vi "VIH Project Tree - Is Drop Allowed.vi"(8 "error in":errorcluster, 9 "Target Item Tag":string, 10 "Source Item Tags":string[](array[string]), 11 "Tree Refnum":refnum<vi>) -> (0 "error out":errorcluster, 1 "Drop Allowed":bool, 3 "dup Tree Refnum":refnum<vi>)   [LabVIEW 2014]
doc: "::: VI Helpeks :::\nCopyright (c) 2000-2026 Konstantin Shifershteyn. All rights reserved."
panel:
  # "VI Helpeks\nCopyright (c) 2012-2026 Konstantin Shifershteyn"
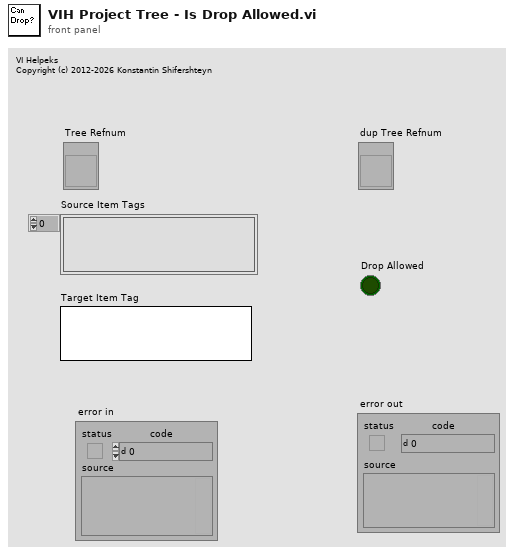
[diagram p1: front panel]
types:
  T1 = typedef "VIH Project Tree Typedef - Tree Item Type.ctl" = enum32{"<Invalid>", "Project", "Proj Files", "Proj Rules", "File Group", "Rule Group", "Any File", "LV Func", ".mnu", ".mnu (dyn)", ".vi", ".vi (dyn)", ".vit", ".vit (dyn)", ".ctl", ".ctl (dyn)", ".ctt", ".ctt (dyn)", "polyVI", "polyVI (dyn)", "expVI", "expVI (dyn)", "HTML", "PolyVI Inst"}
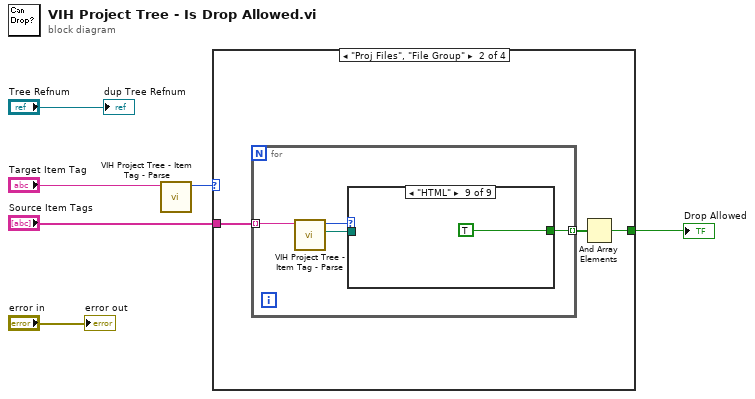
[diagram p0: block diagram]
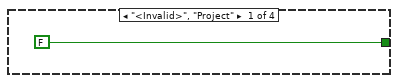
[diagram p2: hidden frame]
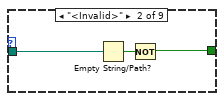
[diagram p4: hidden frame]
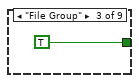
[diagram p5: hidden frame]
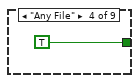
[diagram p6: hidden frame]
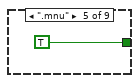
[diagram p7: hidden frame]
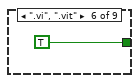
[diagram p8: hidden frame]
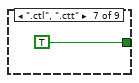
[diagram p9: hidden frame]
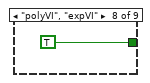
[diagram p10: hidden frame]
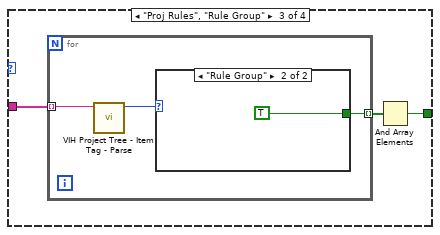
[diagram p11: hidden frame]
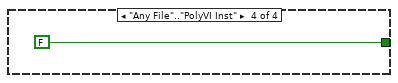
[diagram p13: hidden frame]
diagram:
  n1 = call "VIH Project Tree - Item Tag - Parse.vi"("Tree Item Tag"="Target Item Tag") -> ("Item Type"=w2:T1)  [unwired: 8 in, 2 out]
  n2 = case shown="\"Proj Files\", \"File Group\"" w2 {
    tunnel: [FALSE w9 w26 FALSE] -> w6
    tunnel: "Source Item Tags" -> [_ w8 w25 _]
    frame "<Invalid>", "Project" {
    }
    frame "Proj Files", "File Group" {
      n3 = for {
        tunnel: [w14] -> w10 mode=indexing
        tunnel: w8 -> [w13] mode=indexing
        n4 = call "VIH Project Tree - Item Tag - Parse.vi"("Tree Item Tag"=w13) -> ("Item File Path"=w11:path, "Item Type"=w12:T1)  [unwired: 8 in, 1 out]
        n5 = case shown="\"HTML\"" w12 {
          tunnel: [_ w16 TRUE TRUE TRUE TRUE TRUE TRUE TRUE] -> w14
          tunnel: w11 -> [_ w15 _ _ _ _ _ _ _]
          frame Default {
          }
          frame "<Invalid>" {
            n6 = Empty String/Path?(string/path=w15) -> (empty?=w17:bool)
            n7 = Not(x=w17) -> (.not. x?=w16:bool)
          }
          frame "File Group" {
          }
          frame "Any File" {
          }
          frame ".mnu" {
          }
          frame ".vi", ".vit" {
          }
          frame ".ctl", ".ctt" {
          }
          frame "polyVI", "expVI" {
          }
          frame "HTML" {
          }
        }
      }
      n8 = And Array Elements(Boolean array=w10) -> (logical AND=w9:bool)
    }
    frame "Proj Rules", "Rule Group" {
      n9 = for {
        tunnel: [w30] -> w27 mode=indexing
        tunnel: w25 -> [w29] mode=indexing
        n10 = call "VIH Project Tree - Item Tag - Parse.vi"("Tree Item Tag"=w29) -> ("Item Type"=w28:T1)  [unwired: 8 in, 2 out]
        n11 = case shown="\"Rule Group\"" w28 {
          tunnel: [_ TRUE] -> w30
          frame Default {
          }
          frame "Rule Group" {
          }
        }
      }
      n12 = And Array Elements(Boolean array=w27) -> (logical AND=w26:bool)
    }
    frame "Any File".."PolyVI Inst" {
    }
  }
  "Drop Allowed" <- w6
  "dup Tree Refnum" <- "Tree Refnum"
  "error out" <- "error in"
